vi "Write Scheduled Tx Channel.vi"(4 "Transfer ID map":map{u32, u32}(c390), 6 "data in":u32[](array[numeric]), 7 "disabled transfers":set{u32}(c389), 8 "error in":errorcluster, 9 "labels settings for RT":T1[](array[typedef]) {"Label Timestamp Channel Data Reference" format="%.0x"; "Word Initial Raw Value" format="%032.0f"; "Label Disable/Trigger Channel Reference" format="%.0x"; "parameter driver data"."Tx parameter refs" format="%.0x"; "SDI" format="%02b"; "label" format="%.0o"}, 10 "channel number in":u8, 11 "board handle in":u8) -> (0 "error out":errorcluster, 2 "channel number out":u8, 3 "board handle out":u8, 5 "disabled transfers out":set{u32}(c389))   [LabVIEW 2020, in "AIM ARINC 429 Hardware API.lvlib"]
uses:
  AIM ARINC 429 Hardware API.lvlib
  Shared/RT Label Settings.ctl
  Shared/Label.ctl
  Shared/RT Parameters.ctl
  Shared/Parameter Definition.ctl
  <vilib>/NI/NI VeriStand Encoding and Decoding/Encoding.ctl
  <vilib>/NI VeriStand/Custom Device API/Custom Device Item Ref.ctl
  Shared/Transfer Type.ctl
  <vilib>/NI VeriStand/Custom Device API/Data Reference.ctl
  <instrlib>/AIM GmbH/_ARINC-429/subvi/Error Converter (ErrCode or Status).vi
  <instrlib>/AIM GmbH/_ARINC-429/subvi/Get Library Path.vi
  <instrlib>/AIM GmbH/_ARINC-429/VIs/Library/Api429Lib Error Desc Get.vi
  <instrlib>/AIM GmbH/_ARINC-429/subvi/Get Error Number Offset.vi
  <vilib>/Utility/error.llb/Error Cluster From Error Code.vi
  <instrlib>/AIM GmbH/_ARINC-429/AIM429LV.lvlib
  <vilib>/NI/NI VeriStand Encoding and Decoding/Encoding and Decoding.lvlib
  <vilib>/NI VeriStand/Custom Device API/Custom Device API.lvlib
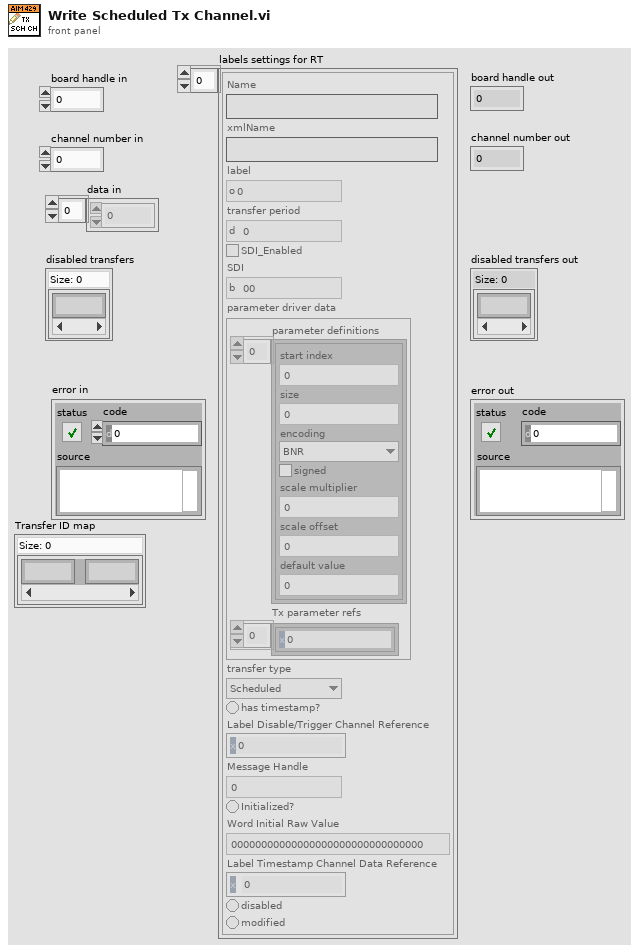
[diagram p1: front panel]
types:
  T1 = typedef "RT Label Settings.ctl" = cluster{"Name":string, "xmlName":string, "label":T2, "transfer period":u32, "SDI_Enabled":bool, "SDI":u8, "parameter driver data":T3, "transfer type":T7, "has timestamp?":bool, "Label Disable/Trigger Channel Reference":T6, "Message Handle":u64, "Initialized?":bool, "Word Initial Raw Value":u32, "Label Timestamp Channel Data Reference":T8, "disabled":bool, "modified":bool}
  T2 = typedef "Label.ctl" = u8
  T3 = typedef "RT Parameters.ctl" = cluster{"parameter definitions":T4[], "Tx parameter refs":T6[]}
  T4 = typedef "Parameter Definition.ctl" = cluster{"start index":i32, "size":i32, "encoding":T5, "signed":bool, "scale multiplier":dbl, "scale offset":dbl, "default value":dbl}
  T5 = typedef "Encoding and Decoding.lvlib/Encoding.ctl" = enum16{"BNR", "BCD", "Discrete"}
  T6 = typedef "Custom Device API.lvlib/Custom Device Item Ref.ctl" = u64
  T7 = typedef "Transfer Type.ctl" = enum16{"Scheduled", "Acyclic", "Block", "Strobe"}
  T8 = typedef "Custom Device API.lvlib/Data Reference.ctl" = i32
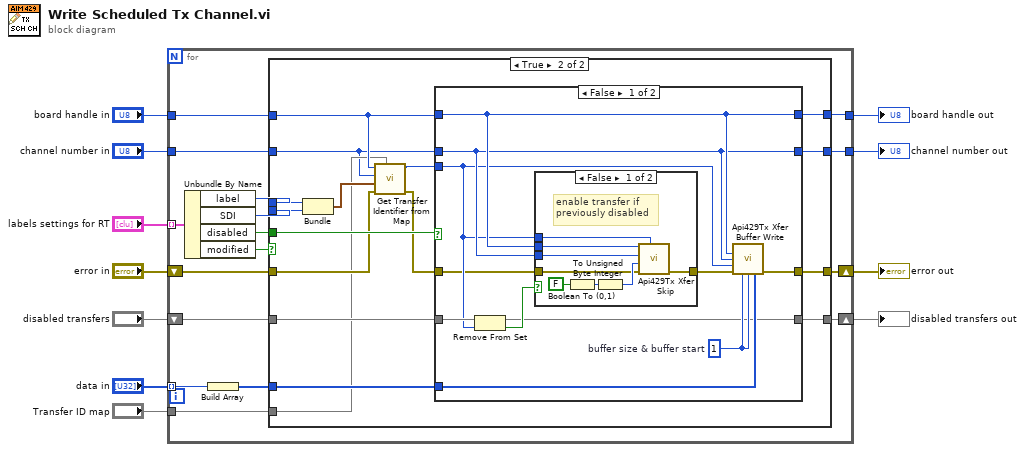
[diagram p0: block diagram]
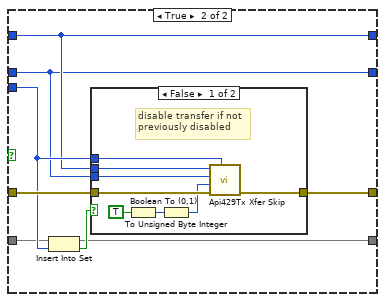
[diagram p4: hidden frame]
diagram:
  n1 = for {
    tunnel: "board handle in" -> [w17]
    tunnel: "channel number in" -> [w16]
    tunnel: "labels settings for RT" -> [w27] mode=indexing
    shift-right: [w24] -> w6
    shift-left: "error in" -> [w18]
    tunnel: "data in" -> [w26] mode=indexing
    tunnel: [w21] -> w5
    tunnel: [w22] -> w4
    shift-right: [w14] -> w2
    shift-left: "disabled transfers" -> [w15]
    tunnel: "Transfer ID map" -> [w12]
    n2 = Unbundle By Name(w27) -> ("label"=w20:T2, "SDI"=w19:u8, "disabled"=w23:bool, "modified"=w13:bool)
    n3 = Build Array(w26) -> (w25:u32[])
    n4 = case shown="True" w13 {
      tunnel: w25 -> [_ w47]
      tunnel: [w29 w46] -> w24
      tunnel: w23 -> [_ w45]
      tunnel: [w31 w44] -> w22
      tunnel: [w30 w43] -> w21
      tunnel: w20 -> [_ w42]
      tunnel: w19 -> [_ w41]
      tunnel: w18 -> [w29 w36]
      tunnel: w17 -> [w31 w38]
      tunnel: w16 -> [w30 w32]
      tunnel: w15 -> [w28 w40]
      tunnel: [w28 w39] -> w14
      tunnel: w12 -> [_ w33]
      frame False {
      }
      frame True {
        n5 = Bundle("label"=w42, "SDI"=w41) -> (w37:cluster{"label":T2, "SDI":u8})  [unwired: 1 in]
        n6 = call "Get Transfer Identifier from Map.vi"("Transfer ID map"=w33, "error in"=w36, "label information"=w37, "channel number in"=w32, "board number in"=w38) -> ("error out"=w35:errorcluster, "Transfer ID out"=w34:u32)  [unwired: 5 in]
        n7 = case shown="False" w45 {
          tunnel: w35 -> [w49 w75]
          tunnel: w47 -> [w57 _]
          tunnel: [w56 w74] -> w46
          tunnel: w32 -> [w51 w68]
          tunnel: w38 -> [w52 w69]
          tunnel: [w52 w69] -> w44
          tunnel: [w51 w68] -> w43
          tunnel: w34 -> [w50 w73]
          tunnel: w40 -> [w55 w72]
          tunnel: [w53 w70] -> w39
          frame False {
            w58 = u16 1  # buffer size & buffer start
            n8 = Remove From Set(10:w50, 11:w55) -> (2:w54:bool, 3:w53:set{u32})
            n9 = case shown="False" w54 {
              tunnel: w52 -> [w66 _]
              tunnel: w51 -> [w65 _]
              tunnel: w50 -> [w64 _]
              tunnel: w49 -> [w60 w67]
              tunnel: [w59 w67] -> w48
              frame False {
                # "enable transfer if\npreviously disabled"
                n10 = Boolean To (0,1)(Boolean=FALSE) -> (0, 1=w62:i16)
                n11 = To Unsigned Byte Integer(number=w62) -> (unsigned 8bit integer=w61:u8)
                n12 = call <instrlib>:"Api429Tx Xfer Skip.vi"("ul_XferId"=w64, "error in (no error)"=w60, "skip"=w61, "b_Chn"=w65, "board_handle"=w66) -> ("error out"=w59:errorcluster)  [unwired: 6 in]
              }
              frame True {
              }
            }
            n13 = call <instrlib>:"Api429Tx Xfer Buffer Write.vi"("board_handle"=w52, "b_Chn"=w51, "ul_XferId"=w50, "error in (no error)"=w48, "w_BufStart"=w58, "w_BufSize"=w58, "pl_LData"=w57) -> ("error out"=w56:errorcluster)  [unwired: 8 in]
          }
          frame True {
            n14 = Insert Into Set(10:w73, 11:w72) -> (2:w71:bool, 3:w70:set{u32})
            n15 = case shown="False" w71 {
              tunnel: w75 -> [w83 w84]
              tunnel: [w77 w84] -> w74
              tunnel: w69 -> [w82 _]
              tunnel: w68 -> [w81 _]
              tunnel: w73 -> [w80 _]
              frame False {
                # "disable transfer if not\npreviously disabled"
                n16 = Boolean To (0,1)(Boolean=TRUE) -> (0, 1=w78:i16)
                n17 = To Unsigned Byte Integer(number=w78) -> (unsigned 8bit integer=w76:u8)
                n18 = call <instrlib>:"Api429Tx Xfer Skip.vi"("ul_XferId"=w80, "error in (no error)"=w83, "skip"=w76, "b_Chn"=w81, "board_handle"=w82) -> ("error out"=w77:errorcluster)  [unwired: 6 in]
              }
              frame True {
                # "do not write data if label is disabled"
              }
            }
          }
        }
      }
    }
  }
  "board handle out" <- w4
  "channel number out" <- w5
  "error out" <- w6
  "disabled transfers out" <- w2
